vi "RemoteVI Retrack Popups.vi"(0 "again?":bool, 1 "popups":T2, 2 "overlay popups":T1(array[cluster]), 3 "popup open?":bool, 5 "panel hWnd":u64, 7 "d":cluster{"dx":i32, "dy":i32}, 9 "remote click?":bool, 10 "popup hWnds":u64[](array[numeric]), 11 "hidden hWnds":u64[](array[numeric])) -> (4 "popups out":T2, 6 "overlay popups out":T1(array[cluster]), 8 "popup open? out":bool, 12 "popup hWnds out":u64[](array[numeric]), 13 "hidden hWnds out":u64[](array[numeric]), 15 "changed?":bool)   [LabVIEW 2020, in "RemoteVI.lvlib"]
doc: "Lists the popups a second time in the same server loop iteration, right after the clients' input was posted (docs\\architecture.md, Popups). When again? is TRUE - a client posted a message that may open a popup (clicked?) or a popup is open (the menu hover may have opened a submenu) - RemoteVI Track Popups.vi runs once more with the outputs of the first listing as previous popup hWnds and previously hidden, so a popup the input just opened is hidden on the host at once instead of one iteration later, and its OVERLAY can go out in this iteration (changed?). When the popups changed it lists again every 25 ms (at most 6 times) until two listings agree: before some menus LabVIEW shows a short-lived window of another size for 30-80 ms (measured), which must not reach the OVERLAY. The WM_NULL round trip after each posted message (RemoteVI Wait Input Handled.vi) has already waited until LabVIEW handled it, so the popup exists by now. Otherwise the first listing is passed through. Win32 only, no VI Server call."
uses:
  RemoteVI.lvlib
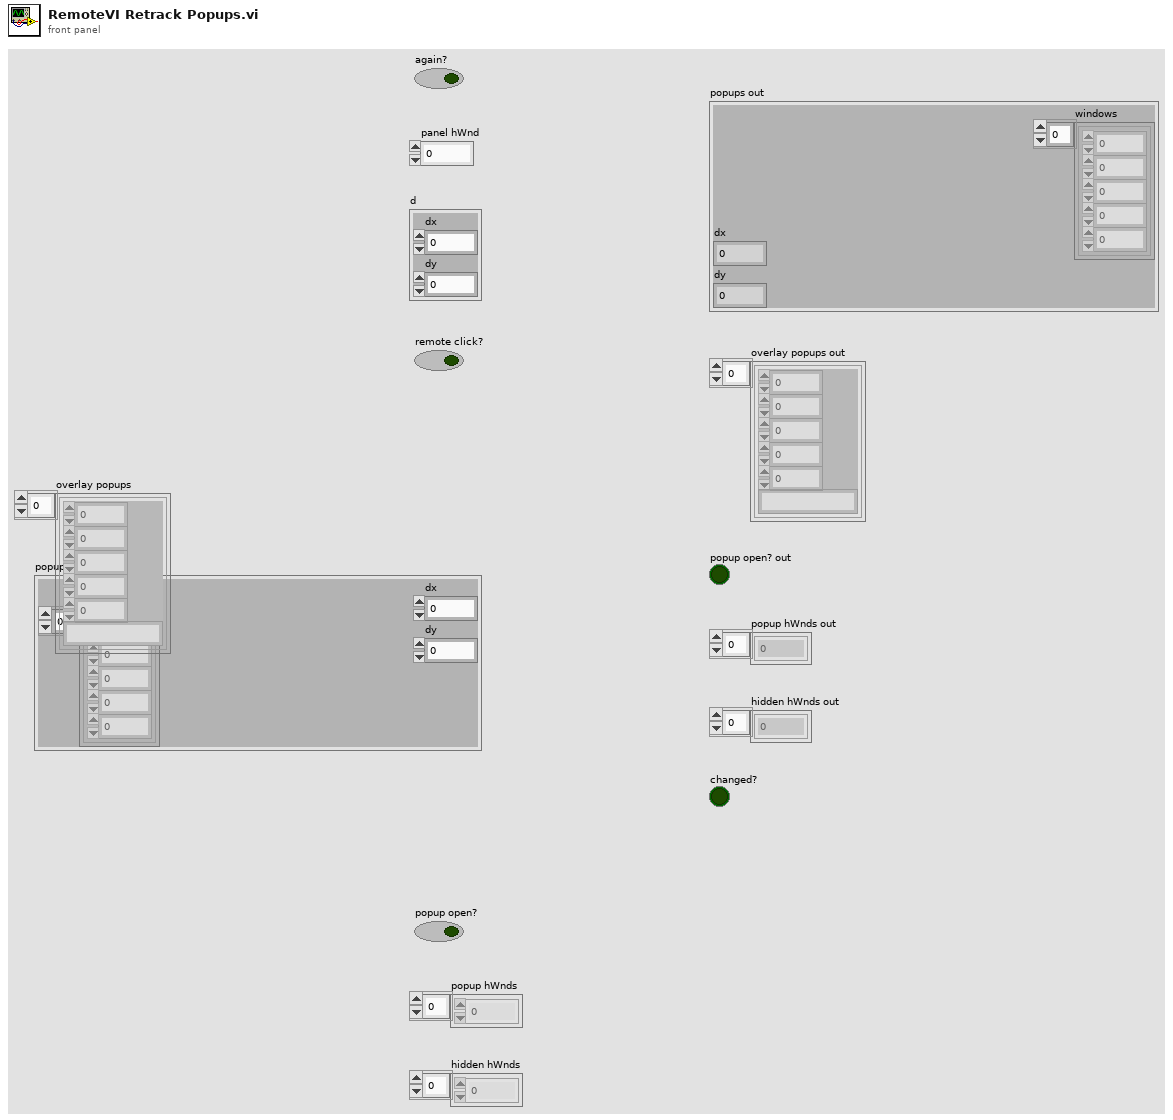
[diagram p1: front panel]
types:
  T1 = cluster{"hwnd":u64, "x":i32, "y":i32, "w":i32, "h":i32, "class":string}[]
  T2 = cluster{"windows":cluster{"hwnd":u64, "x":i32, "y":i32, "w":i32, "h":i32}[], "dx":i32, "dy":i32}
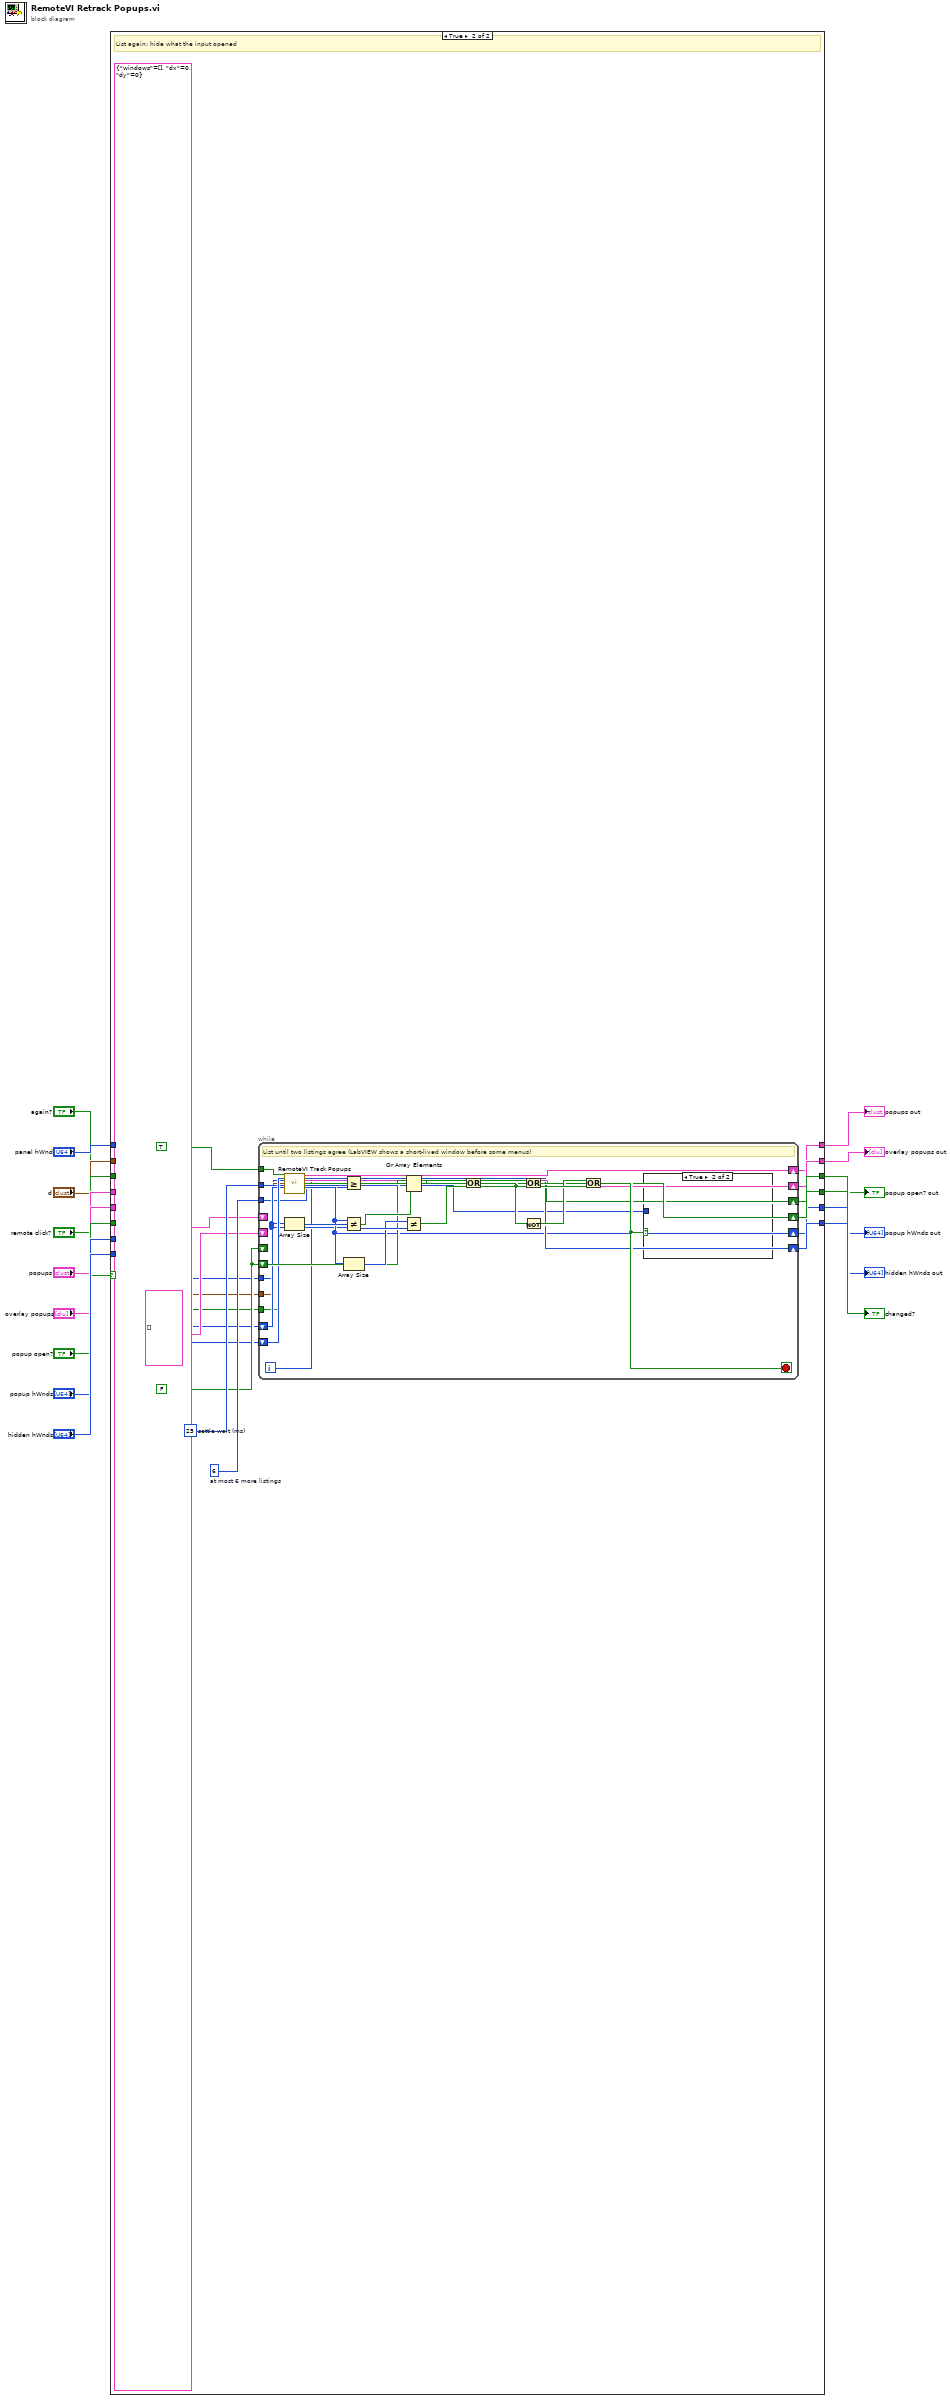
[diagram p0: block diagram]
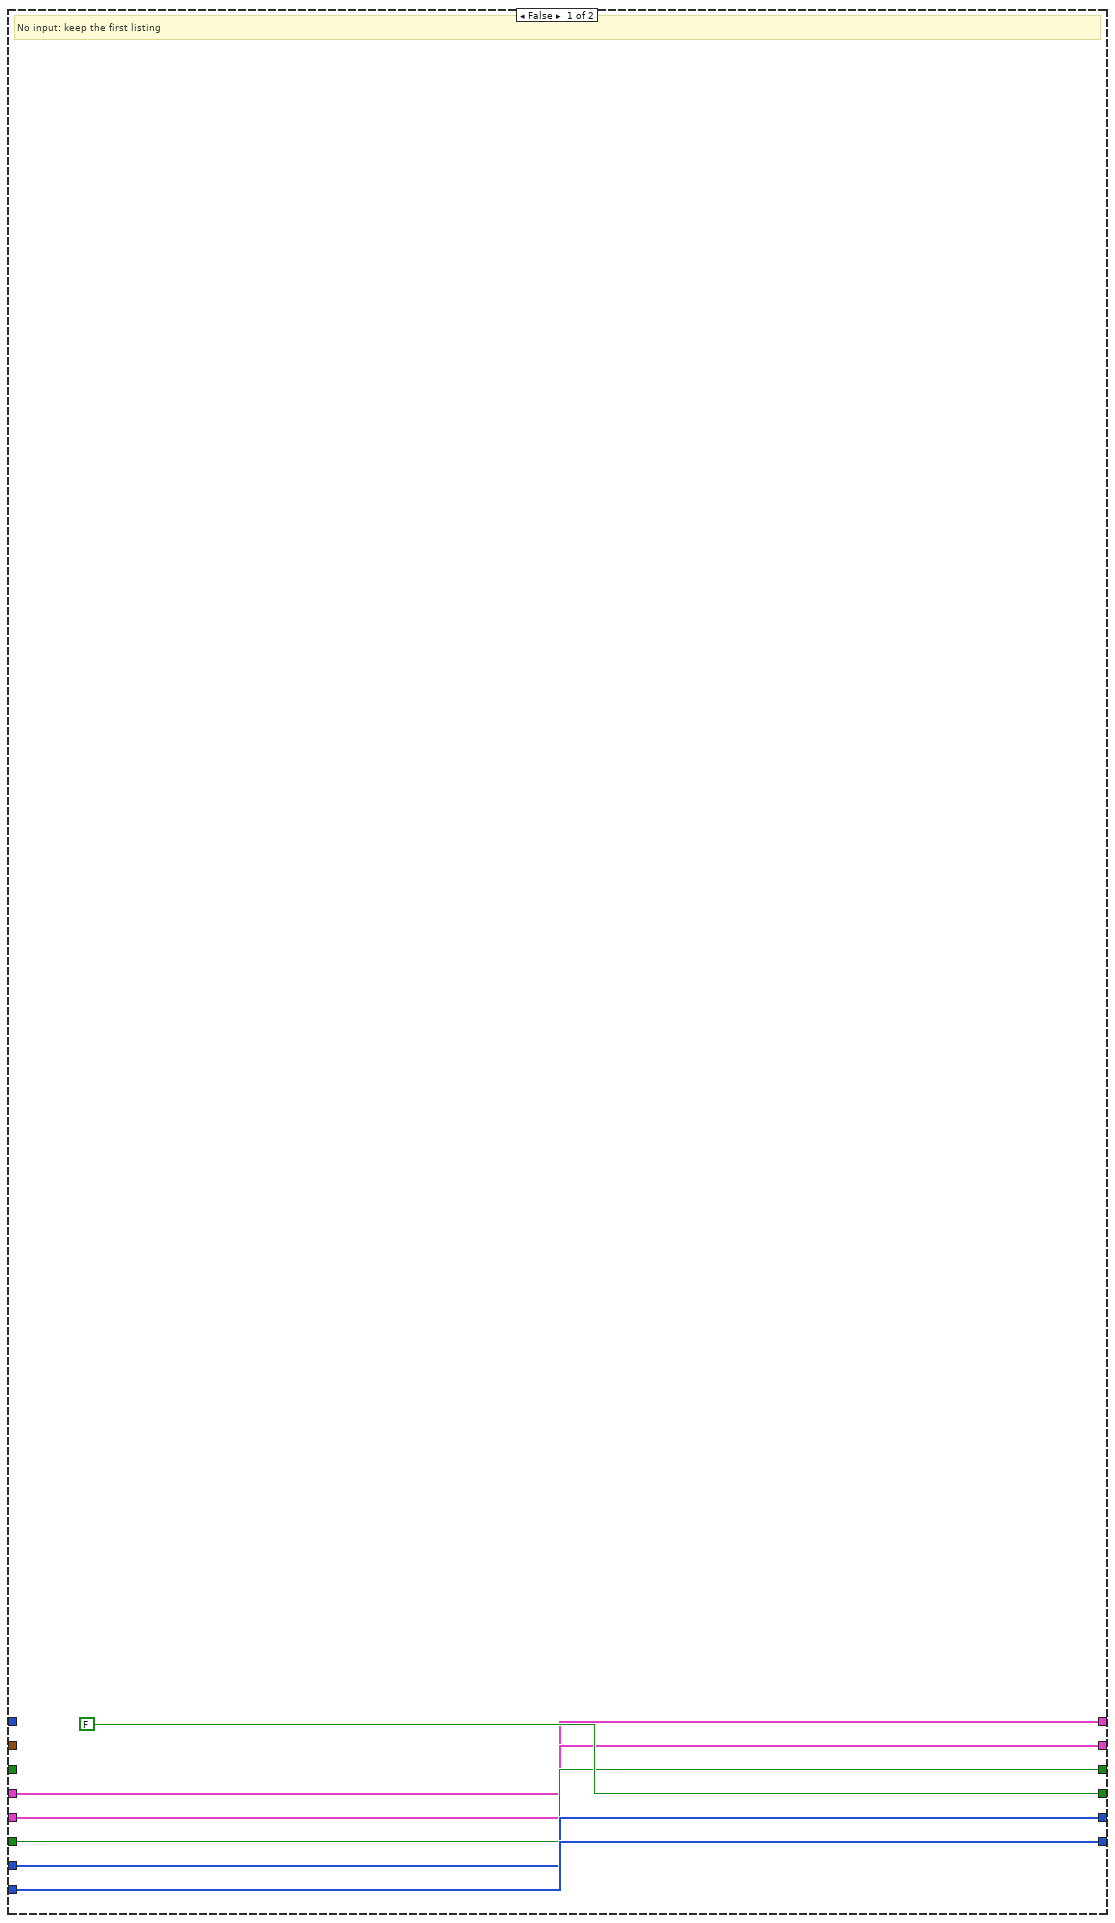
[diagram p2: hidden frame]
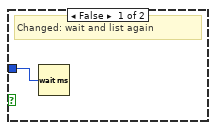
[diagram p3: hidden frame]
diagram:
  n1 = case shown="True" "again?" {
    tunnel: "panel hWnd" -> [_ w22]
    tunnel: "d" -> [_ w23]
    tunnel: "remote click?" -> [_ w24]
    tunnel: "popups" -> [w16 _]
    tunnel: "overlay popups" -> [w17 _]
    tunnel: "popup open?" -> [w18 _]
    tunnel: "popup hWnds" -> [w19 w25]
    tunnel: "hidden hWnds" -> [w20 w26]
    tunnel: [w16 w35] -> w10
    tunnel: [w17 w36] -> w11
    tunnel: [w18 w37] -> w12
    tunnel: [FALSE w38] -> w15
    tunnel: [w19 w33] -> w13
    tunnel: [w20 w34] -> w14
    frame False {
      # "No input: keep the first listing"
    }
    frame True {
      w32 = 6  # at most 6 more listings
      w31 = 25  # settle wait (ms)
      w30 = FALSE
      # "List again: hide what the input opened"
      n2 = while {
        tunnel: TRUE -> [w43]
        tunnel: w31 -> [w44]
        tunnel: w32 -> [w45]
        shift-right: [w50] -> w35
        shift-left: T2 {"windows"=[], "dx"=0, "dy"=0} -> [_]
        shift-right: [w51] -> w36
        shift-left: T1 [] -> [_]
        shift-right: [w52] -> w37
        shift-left: w30 -> [_]
        shift-right: [w54] -> w38
        shift-left: w30 -> [w53]
        tunnel: w22 -> [w40]
        tunnel: w23 -> [w41]
        tunnel: w24 -> [w42]
        shift-right: [w47] -> w33
        shift-left: w25 -> [w46]
        shift-right: [w49] -> w34
        shift-left: w26 -> [w48]
        i -> [w39]
        stop <- w63 stop-if-true
        # "List until two listings agree (LabVIEW shows a short-lived window before some menus)"
        n3 = call "RemoteVI Track Popups.vi"("look?"=w43, "previously hidden"=w48, "remote click?"=w42, "panel hWnd"=w40, "d"=w41, "previous popup hWnds"=w46) -> ("hidden hWnds"=w49:u64[], "popups"=w50:T2, "overlay popups"=w51:T1, "popup open?"=w52:bool, "popup hWnds"=w47:u64[])  [unwired: 5 in]
        n4 = Array Size(array=w46) -> (size(s)=w58:i32)
        n5 = Greater Or Equal?(x=w39, y=w45) -> (x >= y?=w62:bool)
        n6 = Not Equal?(x=w47, y=w46) -> (x != y?=w55:bool[])
        n7 = Array Size(array=w47) -> (size(s)=w57:i32)
        n8 = Or Array Elements(Boolean array=w55) -> (logical OR=w56:bool)
        n9 = Not Equal?(x=w57, y=w58) -> (x != y?=w59:bool)
        n10 = Or(x=w56, y=w59) -> (x .or. y?=w60:bool)
        n11 = Or(x=w53, y=w60) -> (x .or. y?=w54:bool)
        n12 = Not(x=w60) -> (.not. x?=w61:bool)
        n13 = Or(x=w61, y=w62) -> (x .or. y?=w63:bool)
        n14 = case shown="True" w63 {
          tunnel: w44 -> [w64 _]
          frame False {
            # "Changed: wait and list again"
            n15 = Wait (ms)(milliseconds to wait=w64) -> ()  [unwired: 1 out]
          }
          frame True {
          }
        }
      }
    }
  }
  "popups out" <- w10
  "overlay popups out" <- w11
  "popup open? out" <- w12
  "popup hWnds out" <- w13
  "hidden hWnds out" <- w14
  "changed?" <- w15
